vi "Edit Channel.vi"(8 "error in (no error)":errorcluster, 11 "ChannelManagerUI in":refnum<class "ChannelManagerUI.lvclass">) -> (0 "error out":errorcluster, 3 "ChannelManagerUI out":refnum<class "ChannelManagerUI.lvclass">)   [LabVIEW 2021, in "Channel.lvlib" / "ChannelManagerUI.lvlib" / "ChannelManagerUI.lvclass"]
uses:
  ChannelManagerUI.lvclass
  ChannelManagerUI.lvclass/ChannelManagerUI.ctl
  Channel_class/Channel.lvclass
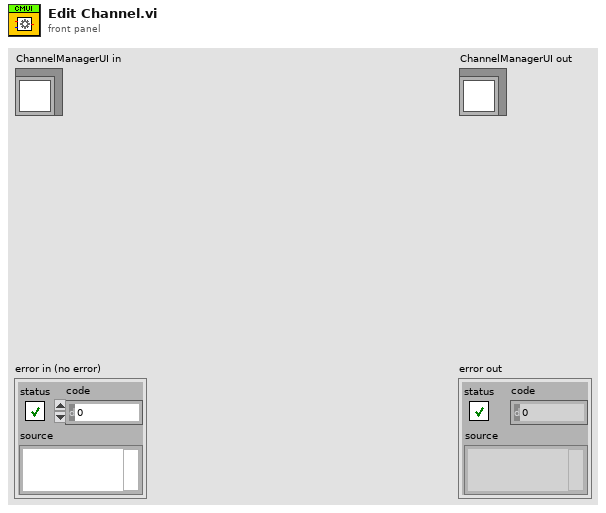
[diagram p1: front panel]
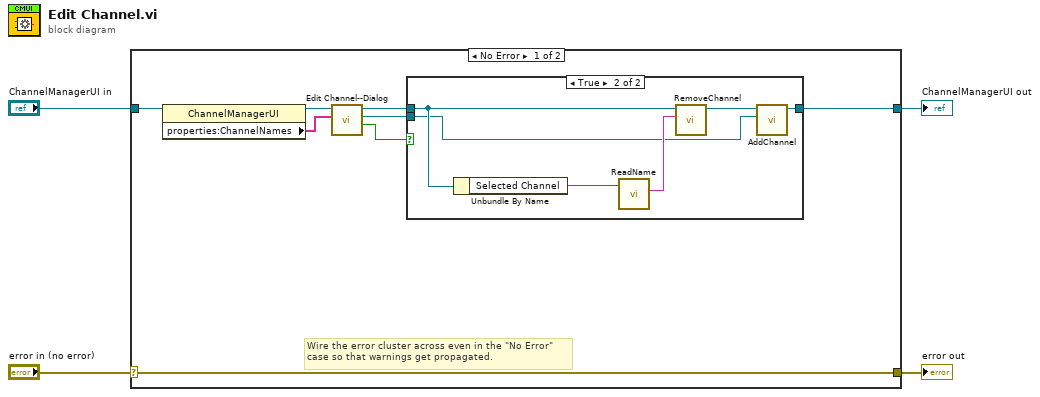
[diagram p0: block diagram]
diagram:
  n1 = case shown="No Error" "error in (no error)" {
    selector: "error in (no error)" -> [w12 w21]
    tunnel: [w12 w21] -> w3
    tunnel: [w8 w20] -> w1
    tunnel: "ChannelManagerUI in" -> [w11 w20]
    frame No Error {
      # "Wire the error cluster across even in the \"No Error\"\ncase so that warnings get propagated."
      n2 = property class="ChannelManagerUI"(reference=w11) -> (reference out=w10:refnum<class "ChannelManagerUI.lvclass">, "properties:ChannelNames"=w9:string[])  [unwired: 1 in, 1 out]
      n3 = call-dynamic "Edit Channel--Dialog.vi"("Channels"=w9, "ChannelManagerUI in"=w10) -> ("OK"=w6:bool, "Class"=w5:refnum<class "Channel.lvclass">, "ChannelManagerUI out"=w7:refnum<class "ChannelManagerUI.lvclass">)  [unwired: 6 in, 1 out]
      n4 = case shown="True" w6 {
        tunnel: [w13 w15] -> w8
        tunnel: w7 -> [w13 w19]
        tunnel: w5 -> [_ w14]
        frame False {
        }
        frame True {
          n5 = Unbundle By Name(w19) -> ("Selected Channel"=w16:refnum<class "Channel.lvclass">)
          n6 = call-dynamic "ReadName.vi"("Channel in"=w16) -> ("Name"=w17:string)  [unwired: 8 in, 2 out]
          n7 = call-dynamic "RemoveChannel.vi"("Name"=w17, "object in"=w19) -> ("object out"=w18:refnum<class "ChannelManagerUI.lvclass">)  [unwired: 8 in, 1 out]
          n8 = call-dynamic "AddChannel.vi"("Channel"=w14, "object in"=w18) -> ("object out"=w15:refnum<class "ChannelManagerUI.lvclass">)  [unwired: 8 in, 1 out]
        }
      }
    }
    frame Error {
    }
  }
  "error out" <- w3
  "ChannelManagerUI out" <- w1
